vi "Neopixel_Indv.vi"(0 "VISA resource name":refnum<visa-resource-name>, 1 "Num_Neo":u8, 2 "Color Box":u32(colorbox), 3 "error in (no error)":errorcluster) -> (7 "VISA resource name out":refnum<visa-resource-name>, 8 "respuesta":string, 10 "error out":errorcluster)   [LabVIEW 2026]
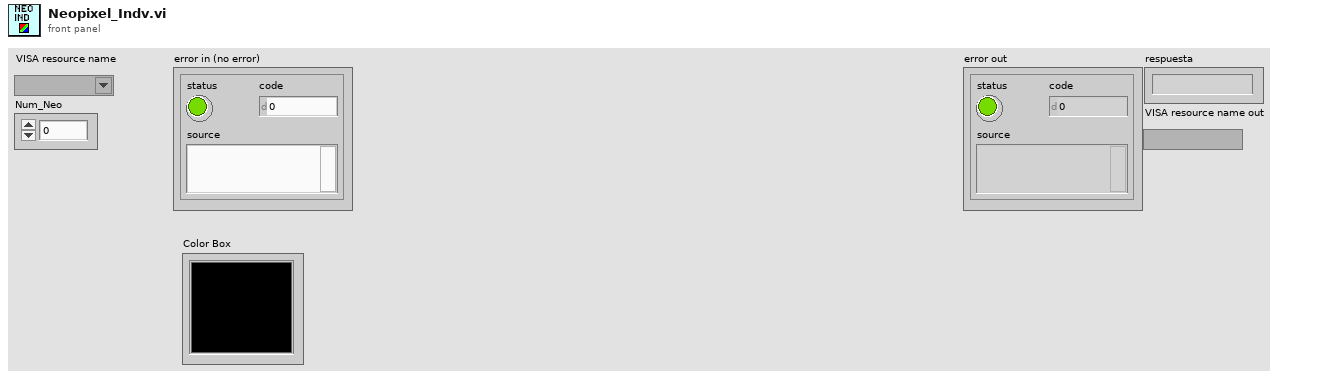
[diagram p1: front panel]
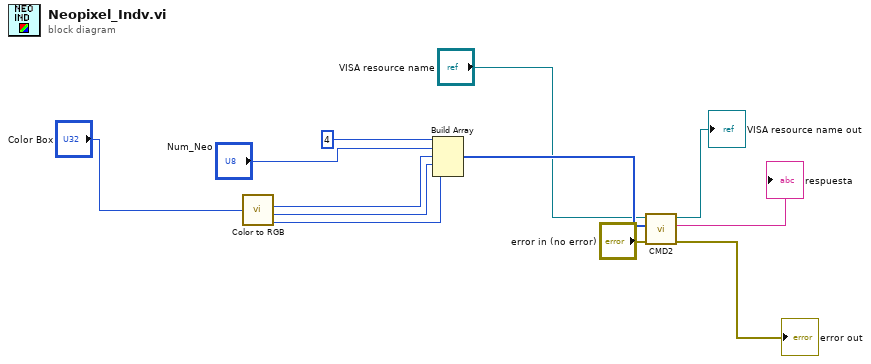
[diagram p0: block diagram]
diagram:
  n1 = call <vilib>:"Color to RGB.vi"("Color"="Color Box") -> ("R"=w11:u8, "G"=w10:u8, "B"=w9:u8)  [unwired: 1 out]
  n2 = Build Array(u8 4, "Num_Neo", w11, w10, w9) -> (w8:u8[])
  n3 = call "CMD2.vi"("error in (no error)"="error in (no error)", "Comando"=w8, "VISA resource name"="VISA resource name") -> ("error out"=→"error out":errorcluster, "respuesta"=→"respuesta":string, "VISA resource name out"=→"VISA resource name out":refnum<visa-resource-name>)  [unwired: 6 in]
